vi "Escape INI String.vi"(8 "error in (no error)":errorcluster, 11 "Text":string) -> (0 "error out":errorcluster, 3 "Escaped":string)   [LabVIEW 2024]
doc: "Escapes a string so it fits on one line of a storage INI file: a backslash is doubled, a line feed becomes backslash-0A and a carriage return backslash-0D - the escapes LabVIEW configuration files use. The caller adds the surrounding double quotes.\n\nGenerated by: Claude"
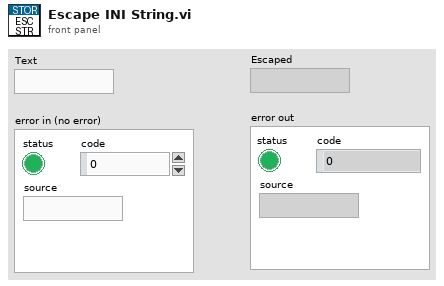
[diagram p1: front panel]
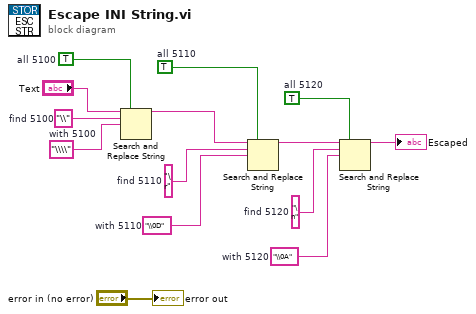
[diagram p0: block diagram]
diagram:
  w13 = TRUE  # all 5120
  w12 = "\\0A"  # with 5120
  w11 = "\n"  # find 5120
  w9 = TRUE  # all 5110
  w8 = "\\0D"  # with 5110
  w7 = "\r"  # find 5110
  w5 = TRUE  # all 5100
  w4 = "\\\\"  # with 5100
  w3 = "\\"  # find 5100
  n1 = Search and Replace String(replace all?=w5, input string="Text", search string=w3, replace string=w4) -> (result string=w6:string)  [unwired: 4 in, 3 out]
  n2 = Search and Replace String(replace all?=w9, input string=w6, search string=w7, replace string=w8) -> (result string=w10:string)  [unwired: 4 in, 3 out]
  n3 = Search and Replace String(replace all?=w13, input string=w10, search string=w11, replace string=w12) -> (result string=→"Escaped":string)  [unwired: 4 in, 3 out]
  "error out" <- "error in (no error)"
